vi "Update Constants.vi"(10 "Subsystem Name":string, 11 "VI in":refnum<vi>) -> (3 "VI out":refnum<vi>)   [LabVIEW 2023]
uses:
  <vilib>/Utility/traverseref.llb/VI Scripting - Traverse.lvlib
  <vilib>/Utility/traverseref.llb/TRef TravTarget.ctl
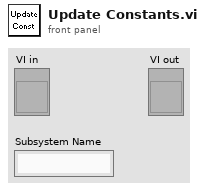
[diagram p1: front panel]
types:
  T1 = typedef "TRef TravTarget.ctl" = enum16{"FP", "BD", "Other"}
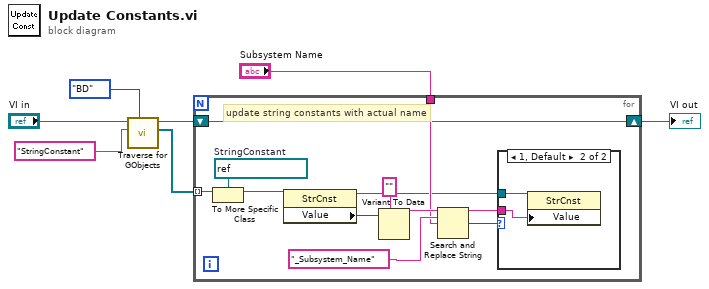
[diagram p0: block diagram]
diagram:
  n1 = call <vilib>:"Traverse for GObjects.vi"("Traverse Target"=TRef_TravTarget."BD", "Class Name"="StringConstant", "VI Refnum"="VI in") -> ("References"=w3:refnum<vi>[], "dup VI Refnum"=w5:refnum<vi>)  [unwired: 5 in, 2 out]
  n2 = for {
    tunnel: w3 -> [w19] mode=indexing
    tunnel: "Subsystem Name" -> [w12]
    shift-right: [w8] -> w6
    shift-left: w5 -> [w8]
    w17 = refnum<vi> refnum  # StringConstant
    # "update string constants with actual name"
    n3 = To More Specific Class(target class=w17, reference=w19) -> (specific class reference=w18:refnum<vi>)  [unwired: 1 in, 1 out]
    n4 = property class="StrCnst"(reference=w18) -> (reference out=w10:refnum<vi>, "Value"=w16:variant)  [unwired: 1 in, 1 out]
    n5 = Variant To Data(type="", Variant=w16) -> (data=w14:string)  [unwired: 1 in, 1 out]
    n6 = Search and Replace String(input string=w14, search string="_Subsystem_Name", replace string=w12) -> (result string=w9:string, number of replacements=w11:i32)  [unwired: 5 in, 2 out]
    n7 = case shown="1, Default" w11 {
      tunnel: w10 -> [_ w21]
      tunnel: w9 -> [_ w20]
      frame 0 {
      }
      frame 1, Default {
        n8 = property class="StrCnst"(reference=w21, "Value"=w20) -> ()  [unwired: 1 in, 2 out]
      }
    }
  }
  "VI out" <- w6
